vi "GetConnectionStatus.vi"(8 "error in (no error)":errorcluster, 11 "object in":refnum<class "DIO_Channel.lvclass">) -> (0 "error out":errorcluster, 2 "Connected?":bool, 3 "object out":refnum<class "DIO_Channel.lvclass">)   [LabVIEW 2021, in "DAQmx.lvlib" / "DIO_Channel.lvclass"]
uses:
  DIO_Channel.lvclass
  DIO_Channel.lvclass/DIO_Channel.ctl
  <vilib>/DAQmx/read.llb/DAQmx Read (Digital Bool 1Line 1Point).vi
  <vilib>/DAQmx/write.llb/DAQmx Write (Digital Bool 1Line 1Point).vi
  DIO-Configuration_class/DIO-Configuration.lvclass
  C:/Users/averna/Documents/LV Gym DEMO/Factory Pattern/Device Channels/Dependencies/DIO-Channel.lvlibp/Channels/DIO-Channel/DIO-Configuration_class/DIO-Configuration.lvclass
  Properties/Get-DIO-DAQmx-Cfg.vi
  <vilib>/DAQmx/miscellaneous.llb/DAQmx Fill In Error Info.vi
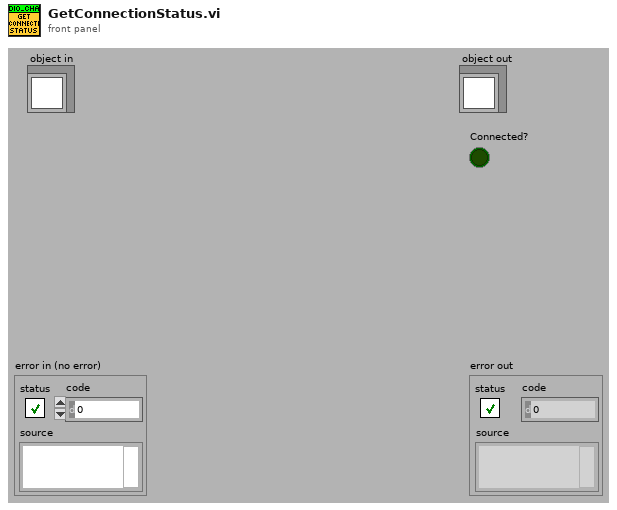
[diagram p1: front panel]
types:
  T1 = typedef "DIO-Channel.lvlibp/DIO-Configuration.lvclass/Direction.ctl" = enum16{"Input", "Output"}
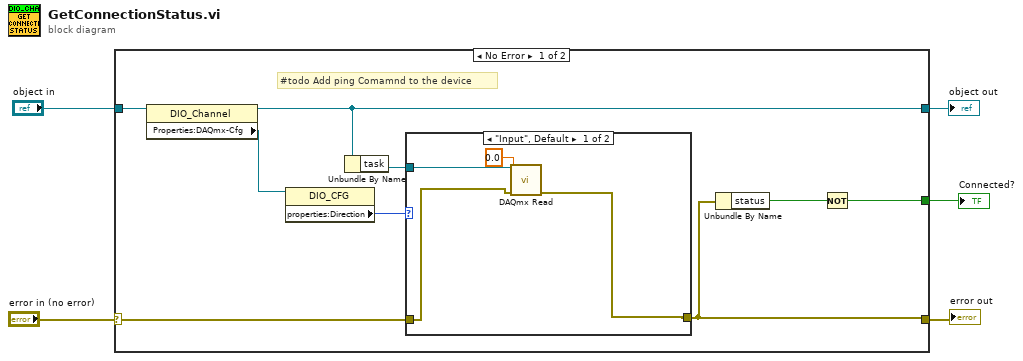
[diagram p0: block diagram]
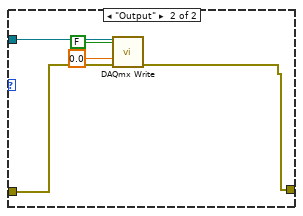
[diagram p2: hidden frame]
diagram:
  n1 = case shown="No Error" "error in (no error)" {
    selector: "error in (no error)" -> [w12 w25]
    tunnel: [w11 w25] -> w4
    tunnel: [w8 w24] -> w2
    tunnel: "object in" -> [w14 w24]
    tunnel: [w9 _] -> w1
    frame No Error {
      # "#todo Add ping Comamnd to the device"
      n2 = property class="DIO_Channel"(reference=w14) -> (reference out=w8:refnum<class "DIO_Channel.lvclass">, "Properties:DAQmx-Cfg"=w7:refnum<class "DIO-Configuration.lvclass">)  [unwired: 1 in, 1 out]
      n3 = property class="DIO_CFG"(reference=w7) -> ("properties:Direction"=w6:T1)  [unwired: 1 in, 2 out]
      n4 = Unbundle By Name(w8) -> ("task"=w13:refnum<k21>)
      n5 = case shown="\"Input\", Default" w6 {
        tunnel: w13 -> [w18 w23]
        tunnel: w12 -> [w17 w22]
        tunnel: [w16 w19] -> w11
        frame "Input", Default {
          n6 = call-poly <vilib>:"DAQmx Read.vi"("task/channels in"=w18, "timeout"=0.0, "error in"=w17) -> ("error out"=w16:errorcluster)  [unwired: 10 in, 2 out]
        }
        frame "Output" {
          n7 = call-poly <vilib>:"DAQmx Write.vi"("task/channels in"=w23, "data"=FALSE, "timeout"=0.0, "error in"=w22) -> ("error out"=w19:errorcluster)  [unwired: 9 in, 2 out]
        }
      }
      n8 = Unbundle By Name(w11) -> ("status"=w10:bool)
      n9 = Not(x=w10) -> (.not. x?=w9:bool)
    }
    frame Error {
    }
  }
  "error out" <- w4
  "object out" <- w2
  "Connected?" <- w1
